vi "set HO Operation Band.vi"(8 "error in (no error)":errorcluster caption="에러 입력(에러 없음)", 9 "Selected CC Argements":T1, 10 "Operation Band":u32, 11 "NR 입력":refnum<class "NR.lvclass">) -> (0 "error out":errorcluster caption="에러 출력", 3 "NR 출력":refnum<class "NR.lvclass">)   [LabVIEW 2023, in "ANRITSU Call Box.lvlib" / "NR.lvclass"]
uses:
  NR.lvclass
  NR.lvclass/NR.ctl
  Type Definition/NR Selected CC Type Arguments.ctl
  ANRITSU Call Box.lvlib
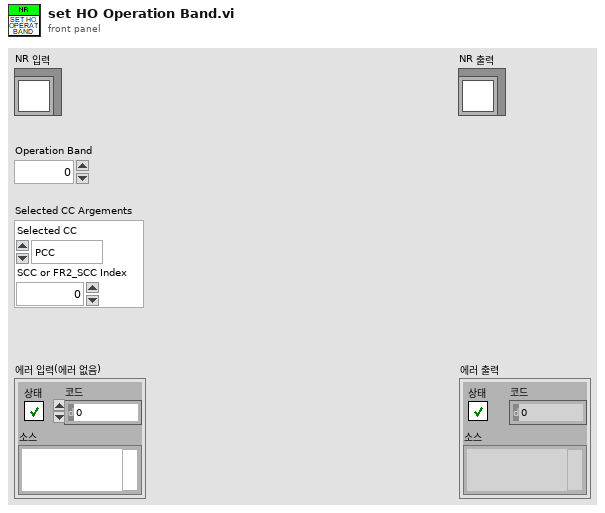
[diagram p1: front panel]
types:
  T1 = typedef "ANRITSU Call Box.lvlib/NR Selected CC Type Arguments.ctl" = cluster{"Selected CC":enum16{"PCC", "SCC", "FR2_PCC", "FR2_SCC"}, "SCC or FR2_SCC Index":u32}
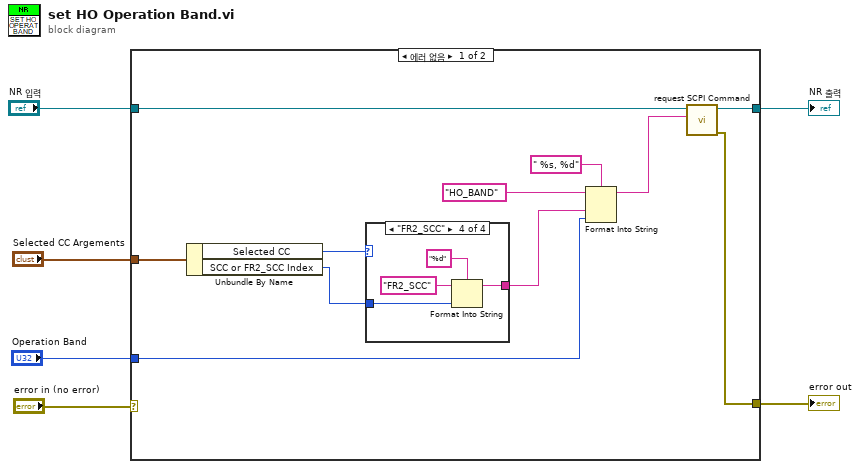
[diagram p0: block diagram]
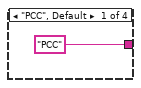
[diagram p2: hidden frame]
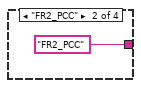
[diagram p3: hidden frame]
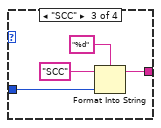
[diagram p4: hidden frame]
diagram:
  n1 = case shown="에러 없음" "error in (no error)" {
    selector: "error in (no error)" -> [_ w29]
    tunnel: [w8 w29] -> w5
    tunnel: [w7 w28] -> w3
    tunnel: "NR 입력" -> [w10 w28]
    tunnel: "Selected CC Argements" -> [w11 _]
    tunnel: "Operation Band" -> [w9 _]
    frame No Error {
      n2 = Unbundle By Name(w11) -> ("Selected CC"=w12:enum16{"PCC", "SCC", "FR2_PCC", "FR2_SCC"}, "SCC or FR2_SCC Index"=w17:u32)
      n3 = case shown="\"FR2_SCC\"" w12 {
        tunnel: ["PCC" "FR2_PCC" w21 w25] -> w14
        tunnel: w17 -> [_ _ w20 w24]
        frame "PCC", Default {
        }
        frame "FR2_PCC" {
        }
        frame "SCC" {
          n4 = Format Into String(format string="%d", initial string="SCC", w20) -> (resulting string=w21:string)  [unwired: 1 in, 1 out]
        }
        frame "FR2_SCC" {
          n5 = Format Into String(format string="%d", initial string="FR2_SCC", w24) -> (resulting string=w25:string)  [unwired: 1 in, 1 out]
        }
      }
      n6 = Format Into String(format string=" %s, %d", initial string="HO_BAND", w14, w9) -> (resulting string=w13:string)  [unwired: 1 in, 1 out]
      n7 = call "request SCPI Command.vi"("SCPI Command"=w13, "NR in"=w10) -> ("error out"=w8:errorcluster, "NR out"=w7:refnum<class "NR.lvclass">)  [unwired: 8 in]
    }
    frame Error {
    }
  }
  "error out" <- w5
  "NR 출력" <- w3
